vi "TCP Server Close Object Reference.vi"(8 "error in (no error)":errorcluster, 11 "TCP Server":refnum<class "JKI TCP Server.lvclass">) -> (0 "error out":errorcluster)   [LabVIEW 2020, in "JKI TCP Server.lvclass"]
uses:
  JKI TCP Server.lvclass
  JKI TCP Server.lvclass/JKI TCP Server.ctl
panel:
  # "<VI NAME>\n\n<DESCRIPTION>\n\nCopyright (C) 2003 Jim Kring jim@jimkring.com\n\nPlease visit http://www.OpenG.org to learn about the\nOpen Source LabVIEW software movement.\n\nThis library is free software; you can redistribute it and/or\nmodify it under the terms of the GNU Lesser General Public\nLicense as published by the Free Software Foundation; either\nversion 2.1 of the License, or (at your option) any later version.\nThis library is distributed in the hope that it will be useful,\nbut WITHOUT ANY WARRANTY; without even the implied warranty of\nMERCHANTABILITY or FITNESS FOR A PARTICULAR PURPOSE. See the GNU\nLesser General Public License for more details.\nYou should have received a copy of the GNU Lesser General Public\nLicense along with this library; if not, write to the Free Software\nFoundation, Inc., 59 Temple Place, Suite 330, Boston, MA 02111-1307 USA"
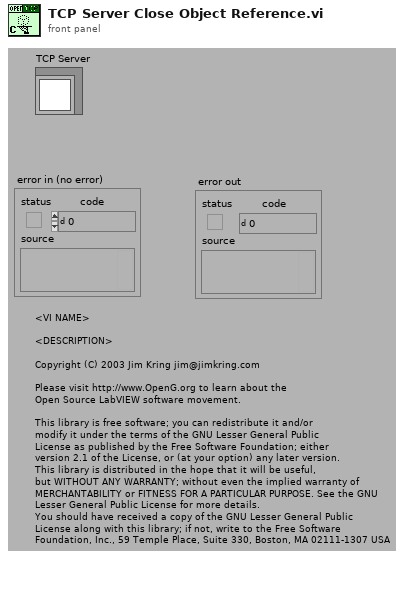
[diagram p1: front panel]
types:
  T1 = typedef "Semaphore RefNum" = refnum<k1>
  T2 = typedef "JKI TCP Server.lvclass/TCP Server Object RefNum.ctl" = refnum<k1>
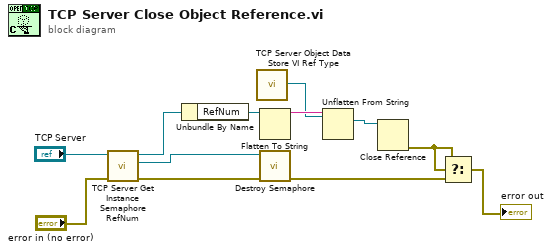
[diagram p0: block diagram]
diagram:
  n1 = call "TCP Server Get Instance Semaphore RefNum.vi"("error out"="error in (no error)", "RefNum"="TCP Server") -> ("error in (no error)"=w7:errorcluster, "semaphore"=w2:T1, "dup RefNum"=w4:refnum<class "JKI TCP Server.lvclass">)  [unwired: 7 in]
  n2 = Unbundle By Name(w4) -> ("RefNum"=w1:T2)
  n3 = call "TCP Server Object Data Store VI Ref Type.vi"() -> ("VI Refnum (Object Data Store.vi Type)"=w5:refnum<vi>)  [unwired: 5 in]
  n4 = Flatten To String(anything=w1) -> (data string=w6:string)  [unwired: 3 in, 2 out]
  n5 = call <vilib>:"Destroy Semaphore.vi"("error in (no error)"=w7, "semaphore"=w2) -> ("error out"=w9:errorcluster)  [unwired: 4 in, 1 out]
  n6 = Unflatten From String(type=w5, binary string=w6) -> (value=w8:refnum<vi>)  [unwired: 3 in, 2 out]
  n7 = Close Reference(reference=w8) -> (error out=w10:errorcluster)  [unwired: 1 in]
  n8 = Select(t=w10, s=w10, f=w9) -> (s? t:f=→"error out":errorcluster)
